vi "SpinCore_API_file_location.vi"() -> ()   [LabVIEW 2024]
panel:
  out "Path":path
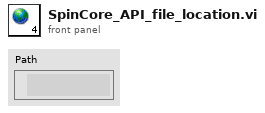
[diagram p1: front panel]
diagram:
